vi "CIF Subscriber to Refnum.vi"(3 "CIF Subscriber U64":u64) -> (5 "CIF Subscriber Refnum":T1 {"refnum" format="%.0x"})   [LabVIEW 2021, in "Iceoryx.lvlib"]
uses:
  Typedef/CIF Subscriber Refnum.ctl
  Iceoryx.lvlib
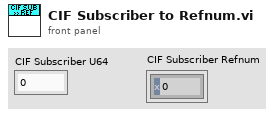
[diagram p1: front panel]
types:
  T1 = typedef "Iceoryx.lvlib/CIF Subscriber Refnum.ctl" = cluster{"refnum":u64, "CIF Sub":enum8{"cifsub"}}
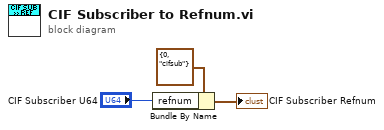
[diagram p0: block diagram]
diagram:
  n1 = Bundle By Name(cluster=T1 {"refnum"=0, "CIF Sub"=enum."cifsub"} ("CIF Subscriber Refnum"), "refnum"="CIF Subscriber U64") -> (→"CIF Subscriber Refnum":T1)
